vi "Update Active VI.vi"(6 "VIWindow":i32, 9 "VIName":string, 10 "Application in":refnum<vi>, 11 "Data in":T1) -> (0 "error out":errorcluster, 1 "Changed?":bool, 2 "Top VI":refnum<class "Standard VI Type.lvclass">, 3 "Data out":T1)   [LabVIEW 2020, in "Peek Window.lvlib"]
uses:
  Peek Window.lvlib
  VI Types/Standard VI Type/Standard VI Type.lvclass
  EHL Data Cluster.ctl
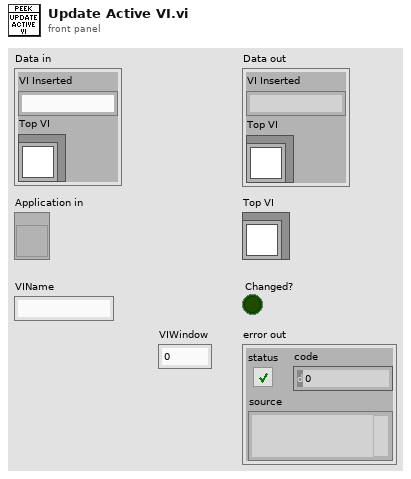
[diagram p1: front panel]
types:
  T1 = typedef "Peek Window.lvlib/EHL Data Cluster.ctl" = cluster{"VI Inserted":string, "Top VI":refnum<class "Standard VI Type.lvclass">}
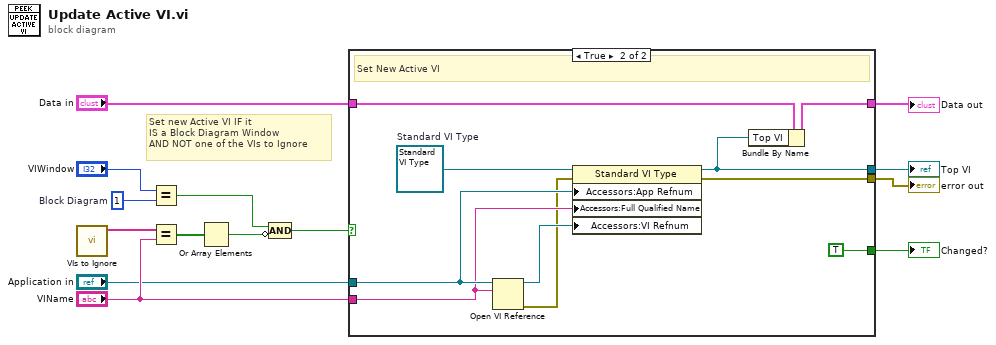
[diagram p0: block diagram]
diagram:
  w6 = 1  # Block Diagram
  # "Set new Active VI IF it\nIS a Block Diagram Window\nAND NOT one of the VIs to Ignore"
  n1 = call "VIs to Ignore.vi"() -> ("VIs to Ignore"=w13:string[])  [unwired: 11 in]
  n2 = Equal?(x="VIWindow", y=w6) -> (x = y?=w5:bool)
  n3 = Equal?(x=w13, y="VIName") -> (x = y?=w9:bool[])
  n4 = Or Array Elements(Boolean array=w9) -> (logical OR=w11:bool)
  n5 = Compound Arithmetic op=AND(w5, invert w11) -> (w8:bool)
  n6 = case shown="True" w8 {
    tunnel: "Application in" -> [_ w20]
    tunnel: "VIName" -> [_ w19]
    tunnel: "Data in" -> [w15 w25]
    tunnel: [w15 w24] -> w4
    tunnel: [_ TRUE] -> w3
    tunnel: [_ w21] -> w2
    tunnel: [_ w16] -> w1
    frame False {
      # "Continue with previous Active VI"
    }
    frame True {
      w22 = refnum<class "Standard VI Type.lvclass"> refnum  # Standard VI Type
      # "Set New Active VI"
      n7 = Open VI Reference(application reference (local)=w20, vi path=w19) -> (vi reference=w18:refnum<vi>, error out=w17:errorcluster)  [unwired: 4 in]
      n8 = property class="Standard VI Type"(reference=w22, error in=w17, "Accessors:App Refnum"=w20, "Accessors:Full Qualified Name"=w19, "Accessors:VI Refnum"=w18) -> (reference out=w21:refnum<class "Standard VI Type.lvclass">, error out=w16:errorcluster)
      n9 = Bundle By Name(cluster=w25, "Top VI"=w21) -> (w24:T1)
    }
  }
  "Data out" <- w4
  "Changed?" <- w3
  "Top VI" <- w2
  "error out" <- w1
